vi "Destroy.vi"(0 "Dashboard Server in":refnum<class "Dashboard Server.lvclass">, 5 "error in (no error)":errorcluster) -> (14 "Dashboard Server out":refnum<class "Dashboard Server.lvclass">, 19 "error out":errorcluster)   [LabVIEW 2019, in "Dashboard Server.lvclass"]
uses:
  Dashboard Server.lvclass
  Dashboard Server.lvclass/Dashboard Server.ctl
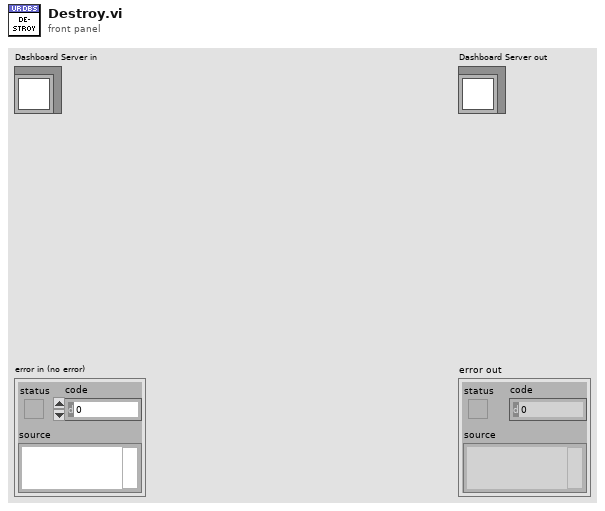
[diagram p1: front panel]
types:
  T1 = typedef "Semaphore RefNum" = refnum<k1>
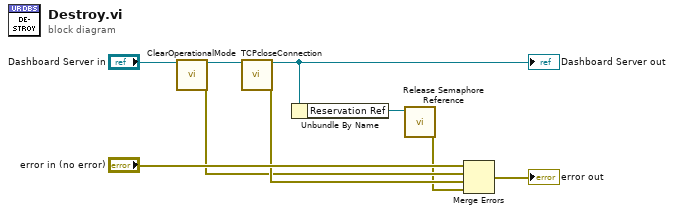
[diagram p0: block diagram]
diagram:
  n1 = call-dynamic "ClearOperationalMode.vi"("DashboardServer in"="Dashboard Server in") -> ("DashboardServer out"=w6:refnum<class "Dashboard Server.lvclass">, "error out"=w4:errorcluster)  [unwired: 16 in, 1 out]
  n2 = call "TCPcloseConnection.vi"("DashboardServer in"=w6) -> ("DashboardServer out"=w3:refnum<class "Dashboard Server.lvclass">, "error out"=w5:errorcluster)  [unwired: 17 in]
  "Dashboard Server out" <- w3
  n3 = Unbundle By Name(w3) -> ("Reservation Ref"=w2:T1)
  n4 = call <vilib>:"Release Semaphore Reference.vi"("semaphore"=w2) -> ("error out"=w1:errorcluster)  [unwired: 9 in, 1 out]
  n5 = Merge Errors("error in (no error)", w4, w5, w1) -> (→"error out":errorcluster)
